vi "Get Variable Container.vi"(8 "error in (no error)":errorcluster, 10 "Type":T2, 11 "TSEngine in":refnum<class "Engine.lvclass">) -> (0 "error out":errorcluster, 2 "VariableContainer":T1, 3 "TSEngine out":refnum<class "Engine.lvclass">)   [LabVIEW 2020, in "TSS.lvlib" / "Engine.lvclass"]
uses:
  Engine.lvclass
  Variable Container Type.ctl
  VariableContainer/Typedefs/Session Handle.ctl
  VariableContainer/VariableContainer.lvclass
  Create VC Event Data.ctl
  Engine.lvclass/Engine.ctl
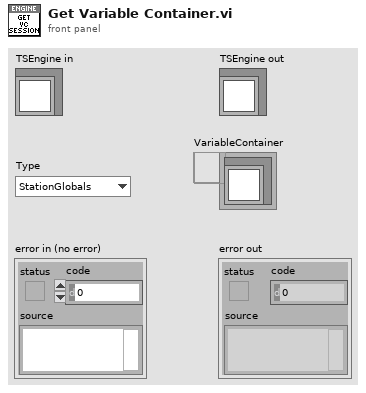
[diagram p1: front panel]
types:
  T1 = typedef "TSS.lvlib/VariableContainer.lvclass/Session Handle.ctl" = refnum<data-value>
  T2 = typedef "TSS.lvlib/Engine.lvclass/Variable Container Type.ctl" = enum16{"StationGlobals", "TemporaryGlobals", "NewPropertyObject"}
  T3 = typedef "TSS.lvlib/Engine.lvclass/Create VC Event Data.ctl" = cluster{"Type":T2, "Notifier":refnum<notifier>}
  T4 = typedef "TSS.lvlib/Engine.lvclass/Events.ctl" = cluster{"Stop Deamon":refnum<user-event>, "Create Variable Container":refnum<user-event>, "Create Report":refnum<user-event>, "Open Sequence File":refnum<user-event>, "Prepare Execution":refnum<user-event>}
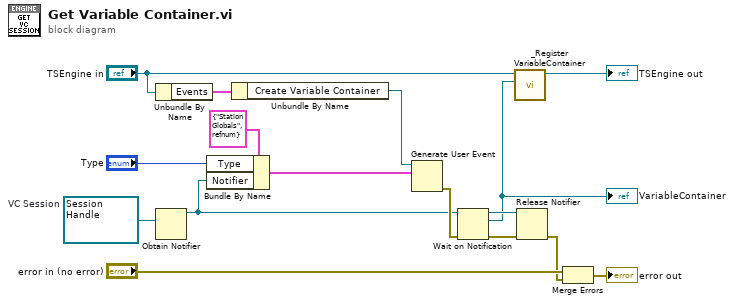
[diagram p0: block diagram]
diagram:
  w15 = T1 refnum  # VC Session
  n1 = Unbundle By Name("TSEngine in") -> ("Events"=w5:T4)
  n2 = Obtain Notifier(notification data type=w15) -> (notifier out=w12:refnum<notifier>)  [unwired: 3 in, 2 out]
  n3 = Bundle By Name(cluster=T3 {"Type"=enum."StationGlobals", "Notifier"=refnum} ("Create Session Event Data"), "Type"="Type", "Notifier"=w12) -> (w11:T3)
  n4 = Unbundle By Name(w5) -> ("Create Variable Container"=w4:refnum<user-event>)
  n5 = Generate User Event(user event=w4, event data cluster=w11) -> (error out=w16:errorcluster)  [unwired: 2 in, 1 out]
  n6 = Wait on Notification(notifier=w12, error in (no error)=w16) -> (notifier out=w9:refnum<notifier>, notification=w1:T1, error out=w8:errorcluster)  [unwired: 2 in, 1 out]
  "VariableContainer" <- w1
  n7 = call "_Register VariableContainer.vi"("VariableContainer"=w1, "Engine in"="TSEngine in") -> ("Engine out"=→"TSEngine out":refnum<class "Engine.lvclass">)  [unwired: 8 in, 1 out]
  n8 = Release Notifier(notifier=w9, error in (no error)=w8) -> (error out=w6:errorcluster)  [unwired: 1 in, 2 out]
  n9 = Merge Errors("error in (no error)", w6) -> (→"error out":errorcluster)
